vi "RemoteVI WS Decode Client Frame.vi"(0 "buffer":string, 1 "max payload":u32=65536) -> (14 "complete?":bool, 15 "fin":bool, 16 "opcode":u8, 17 "payload":string, 18 "bytes consumed":u32, 19 "close code":u16)   [LabVIEW 2020, in "RemoteVI.lvlib"]
doc: "Decodes one masked client-to-server WebSocket frame (RFC 6455) from the start of buffer. complete? is FALSE with close code 0 when more bytes are needed. A protocol violation gives complete? FALSE and close code 1002 (RSV bits set, unknown opcode, unmasked frame, control frame over 125 bytes or fragmented) or 1009 (payload longer than max payload). On success the unmasked payload is returned and bytes consumed is the frame size to drop from the buffer. Pure function. Reference: decodeClientFrame() in tools\\lib\\websocket.mjs."
uses:
  RemoteVI.lvlib
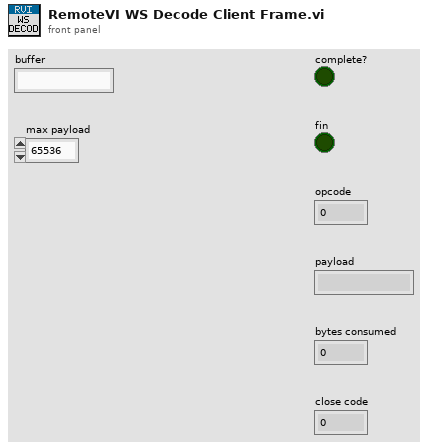
[diagram p1: front panel]
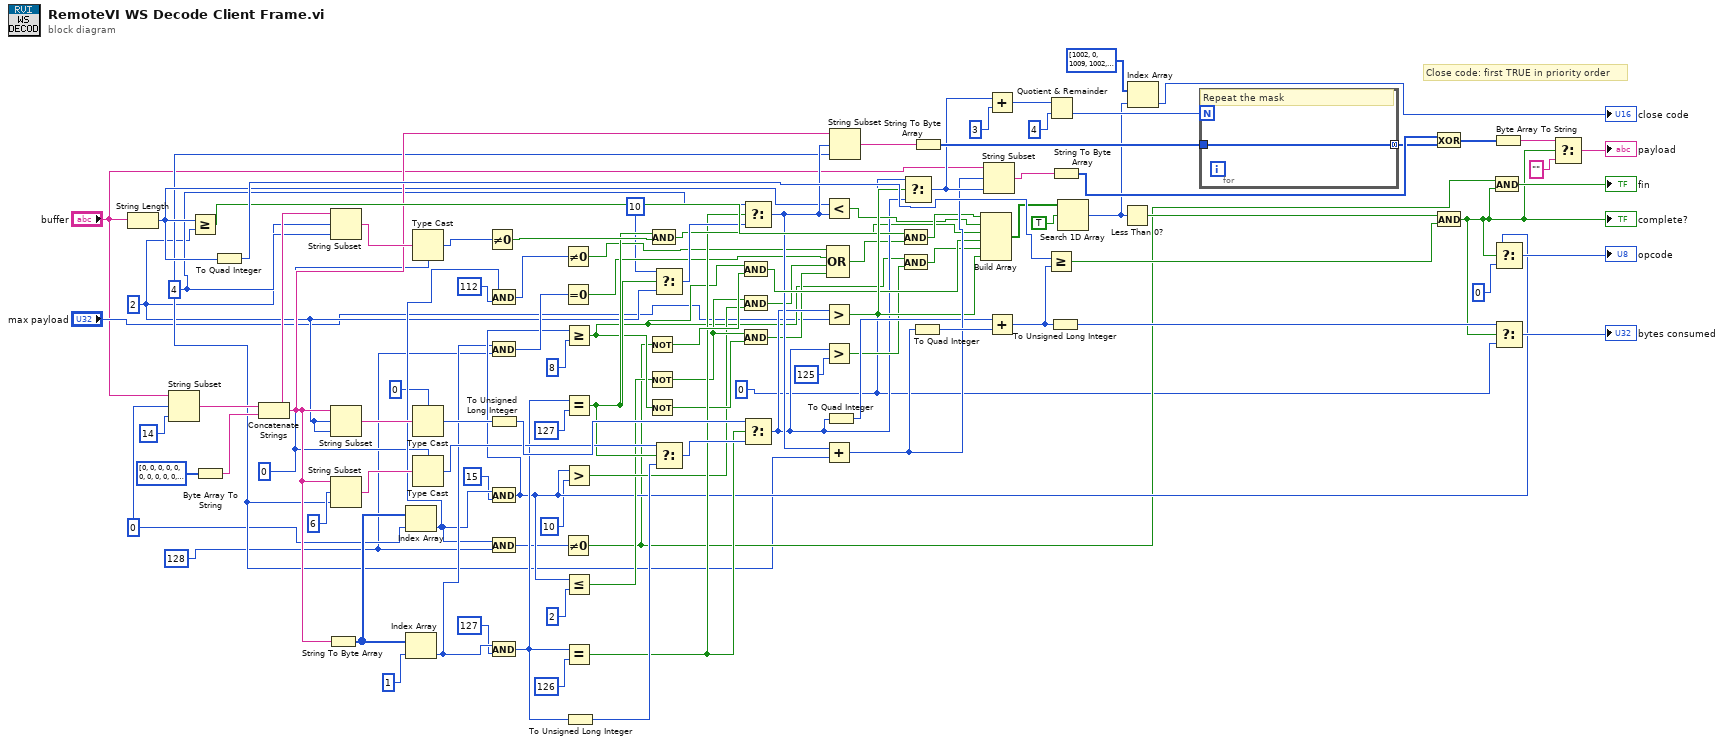
[diagram p0: block diagram]
diagram:
  w22 = u32 0
  w20 = u32 0
  w16 = 4
  w15 = 2
  w13 = 0
  w3 = u8 128
  # "Close code: first TRUE in priority order"
  n1 = String Length(string="buffer") -> (length=w30:i32)
  n2 = String Subset(string="buffer", offset (0)=w13, length (rest)=14) -> (substring=w31:string)
  n3 = Greater Or Equal?(x=w30, y=w15) -> (x >= y?=w69:bool)
  n4 = Byte Array To String(unsigned byte array=u8[] [0, 0, 0, 0, 0, 0, 0, 0, 0, 0, 0, 0, 0, 0]) -> (string=w32:string)
  n5 = To Quad Integer(1:w30) -> (0:w84:i64)
  n6 = Concatenate Strings(w31, w32) -> (w33:string)
  n7 = String To Byte Array(string=w33) -> (unsigned byte array=w34:u8[])
  n8 = String Subset(string=w33, offset (0)=w15, length (rest)=w16) -> (substring=w57:string)
  n9 = String Subset(string=w33, offset (0)=w15, length (rest)=w15) -> (substring=w55:string)
  n10 = String Subset(string=w33, offset (0)=6, length (rest)=w16) -> (substring=w61:string)
  n11 = Index Array(array=w34, index=w13) -> (element=w35:u8)
  n12 = Index Array(array=w34, index=1) -> (element=w36:u8)
  n13 = Type Cast(type=w22, x=w57) -> (*(type *) &x=w58:u32)
  n14 = Type Cast(type=u16 0, x=w55) -> (*(type *) &x=w56:u16)
  n15 = Type Cast(type=w22, x=w61) -> (*(type *) &x=w62:u32)
  n16 = Not Equal To 0?(x=w58) -> (x != 0?=w59:bool)
  n17 = And(x=w35, y=u8 112) -> (x .and. y?=w39:u8)
  n18 = And(x=w36, y=w3) -> (x .and. y?=w42:u8)
  n19 = To Unsigned Long Integer(number=w56) -> (unsigned 32bit integer=w63:u32)
  n20 = And(x=w35, y=u8 15) -> (x .and. y?=w41:u8)
  n21 = And(x=w35, y=w3) -> (x .and. y?=w37:u8)
  n22 = And(x=w36, y=u8 127) -> (x .and. y?=w44:u8)
  n23 = Not Equal To 0?(x=w39) -> (x != 0?=w40:bool)
  n24 = Equal To 0?(x=w42) -> (x = 0?=w43:bool)
  n25 = Not Equal To 0?(x=w37) -> (x != 0?=w38:bool)
  n26 = Greater Or Equal?(x=w41, y=u8 8) -> (x >= y?=w46:bool)
  n27 = Equal?(x=w44, y=u8 127) -> (x = y?=w54:bool)
  n28 = Greater?(x=w41, y=u8 10) -> (0:w47:bool)
  n29 = Less Or Equal?(x=w41, y=u8 2) -> (x <= y?=w45:bool)
  n30 = Equal?(x=w44, y=u8 126) -> (x = y?=w53:bool)
  n31 = To Unsigned Long Integer(number=w44) -> (unsigned 32bit integer=w64:u32)
  n32 = Not(x=w38) -> (.not. x?=w73:bool)
  n33 = Not(x=w45) -> (.not. x?=w48:bool)
  n34 = Not(x=w46) -> (.not. x?=w50:bool)
  n35 = And(x=w54, y=w59) -> (x .and. y?=w60:bool)
  n36 = Select(t=10, s=w54, f=w15) -> (s? t:f=w67:i32)
  n37 = Select(t=w62, s=w54, f=w64) -> (s? t:f=w65:u32)
  n38 = And(x=w46, y=w73) -> (x .and. y?=w75:bool)
  n39 = And(x=w48, y=w47) -> (x .and. y?=w49:bool)
  n40 = And(x=w48, y=w50) -> (x .and. y?=w51:bool)
  n41 = Select(t=w16, s=w53, f=w67) -> (s? t:f=w68:i32)
  n42 = Select(t=w63, s=w53, f=w65) -> (s? t:f=w66:u32)
  n43 = Less?(x=w30, y=w68) -> (x < y?=w70:bool)
  n44 = Greater?(x=w66, y="max payload") -> (0:w76:bool)
  n45 = Greater?(x=w66, y=u32 125) -> (0:w72:bool)
  n46 = Add(x=w68, y=w16) -> (x+y=w81:i32)
  n47 = To Quad Integer(1:w66) -> (0:w80:i64)
  n48 = Compound Arithmetic op=OR(w40, w43, w49, w51) -> (w52:bool)
  n49 = String Subset(string=w33, offset (0)=w68, length (rest)=w16) -> (substring=w90:string)
  n50 = And(x=w69, y=w52) -> (x .and. y?=w71:bool)
  n51 = And(x=w46, y=w72) -> (x .and. y?=w74:bool)
  n52 = Select(t=w20, s=w76, f=w66) -> (s? t:f=w88:u32)
  n53 = To Quad Integer(1:w81) -> (0:w82:i64)
  n54 = String To Byte Array(string=w90) -> (unsigned byte array=w91:u8[])
  n55 = Build Array(w71, w70, w60, w75, w74, w76) -> (w77:bool[])
  n56 = String Subset(string="buffer", offset (0)=w81, length (rest)=w88) -> (substring=w89:string)
  n57 = Add(x=w88, y=u32 3) -> (x+y=w92:u32)
  n58 = Add(x=w80, y=w82) -> (x+y=w83:i64)
  n59 = Greater Or Equal?(x=w84, y=w83) -> (x >= y?=w85:bool)
  n60 = Quotient & Remainder(x=w92, y=u32 4) -> (floor(x/y)=w93:u32)  [unwired: 1 out]
  n61 = To Unsigned Long Integer(number=w83) -> (unsigned 32bit integer=w99:u32)
  n62 = String To Byte Array(string=w89) -> (unsigned byte array=w95:u8[])
  n63 = Search 1D Array(1D array=w77, element=TRUE) -> (index of element=w78:i32)  [unwired: 1 in]
  n64 = Less Than 0?(x=w78) -> (x < 0?=w86:bool)
  n65 = Index Array(array=u16[] [1002, 0, 1009, 1002, 1002, 1009], index=w78) -> (element=→"close code":u16)
  n66 = for {
    N: w93 -> [_]
    tunnel: w91 -> [w103]
    tunnel: [w103] -> w94 mode=concatenating
    # "Repeat the mask"
  }
  n67 = Exclusive Or(1:w94, 2:w95) -> (0:w96:u8[])
  n68 = And(x=w86, y=w85) -> (x .and. y?=w87:bool)
  "complete?" <- w87
  n69 = And(x=w38, y=w87) -> (x .and. y?=→"fin":bool)
  n70 = Byte Array To String(unsigned byte array=w96) -> (string=w97:string)
  n71 = Select(t=w41, s=w87, f=u8 0) -> (s? t:f=→"opcode":u8)
  n72 = Select(t=w99, s=w87, f=w20) -> (s? t:f=→"bytes consumed":u32)
  n73 = Select(t=w97, s=w87, f="") -> (s? t:f=→"payload":string)
